vi "IRread.vi"(2 "error in (no error)":errorcluster, 3 "AI Ref In":T2) -> (0 "error out":errorcluster, 1 "紅外線數值":T1)   [LabVIEW 2019]
uses:
  <vilib>/myRIO/Instrument Drivers/Onboard IO/AI/typedefs/AI Reference.ctl
  <vilib>/myRIO/Common/Instrument Driver Framework/Utilities/typedefs/myRIO Generic Hardware Reference.ctl
  <vilib>/myRIO/Common/Instrument Driver Framework/Utilities/typedefs/Hardware Version Enum.ctl
  <vilib>/myRIO/Common/Instrument Driver Framework/Utilities/typedefs/myRIO v1.0 Reference.ctl
  <vilib>/myRIO/Common/Instrument Driver Framework/Utilities/typedefs/Generic FPGA Reference.ctl
  <vilib>/myRIO/Common/Instrument Driver Framework/myRIO v1.0/AI/typedefs/AI Channels List.ctl
  <vilib>/myRIO/Common/Instrument Driver Framework/myRIO v1.0/AI/typedefs/AI Channels Enum.ctl
  <vilib>/myRIO/Common/Instrument Driver Framework/Utilities/typedefs/Analog Scaling Constants List.ctl
  <vilib>/myRIO/Common/Instrument Driver Framework/Utilities/typedefs/Analog Scaling Constants.ctl
  <vilib>/Utility/error.llb/Error Cluster From Error Code.vi
  <vilib>/myRIO/Common/Instrument Driver Framework/myRIO v1.0/AI/vis/myRIO v1.0 Read AI.vi
  <vilib>/myRIO/Instrument Drivers/Onboard IO/AI/AI.lvlib
  <vilib>/ptbypt/NI_PtbyPt.lvlib
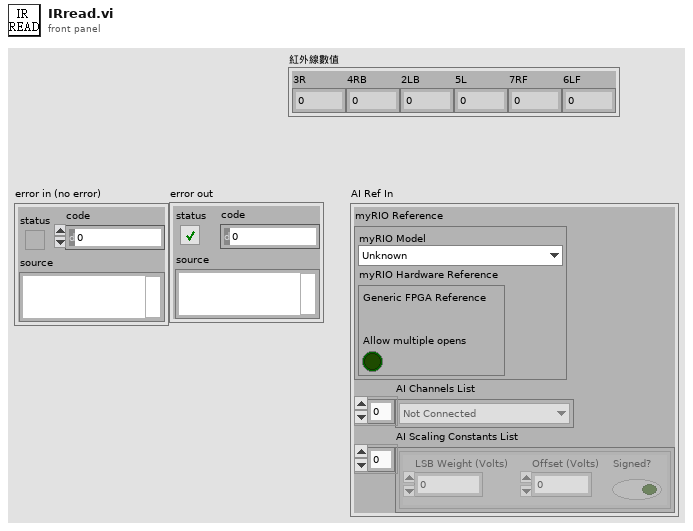
[diagram p1: front panel]
types:
  T1 = cluster{"7RF":dbl, "3R":dbl, "4RB":dbl, "5L":dbl, "6LF":dbl, "2LB":dbl}
  T2 = typedef "AI.lvlib/AI Reference.ctl" = cluster{"myRIO Reference":T3, "AI Channels List":T7, "AI Scaling Constants List":T9}
  T3 = typedef "myRIO Generic Hardware Reference.ctl" = cluster{"myRIO Model":T4, "myRIO Hardware Reference":T5}
  T4 = typedef "Hardware Version Enum.ctl" = enum16{"Unknown", "myRIO-1900", "myRIO-1950", "roboRIO", "NI ELVIS RIO CM", "ELVIS III"}
  T5 = typedef "myRIO v1.0 Reference.ctl" = cluster{"Generic FPGA Reference":T6, "Allow multiple opens":bool}
  T6 = typedef "Generic FPGA Reference.ctl" = refnum<k20>
  T7 = typedef "AI Channels List.ctl" = T8[]
  T8 = typedef "AI Channels Enum.ctl" = enum16{"Not Connected", "AudioIn/Left", "AudioIn/Right", "C/AI0", "C/AI1", "A/AI0", "A/AI1", "A/AI2", "A/AI3", "A/AI4", "A/AI5", "A/AI6", "A/AI7", "B/AI0", "B/AI1", "B/AI2", "B/AI3", "B/AI4", "B/AI5", "B/AI6", "B/AI7", "AI/AI0", "AI/AI1", "AI/AI2", "AI/AI3", "A/AI0 (DIFF)", "A/AI1 (DIFF)", "A/AI2 (DIFF)", "A/AI3 (DIFF)", "B/AI0 (DIFF)", "B/AI1 (DIFF)", "B/AI2 (DIFF)", "B/AI3 (DIFF)"}
  T9 = typedef "Analog Scaling Constants List.ctl" = T10[]
  T10 = typedef "Analog Scaling Constants.ctl" = cluster{"LSB Weight (Volts)":dbl, "Offset (Volts)":dbl, "Signed?":bool}
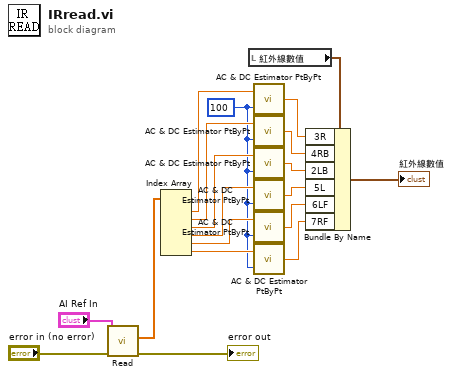
[diagram p0: block diagram]
diagram:
  w1 = 100 ("sample length")
  n1 = call <vilib>:"Read.vi"("error in (no error)"="error in (no error)", "AI Ref In"="AI Ref In") -> ("error out"=→"error out":errorcluster, "Values"=w18:dbl[])  [unwired: 7 in, 1 out]
  n2 = Index Array(array=w18) -> (element #1=w13:dbl, element #2=w12:dbl, element #3=w11:dbl, element #4=w10:dbl, element #5=w9:dbl, element #6=w8:dbl)  [unwired: 6 in]
  n3 = local read "紅外線數值"() -> (w14:T1)
  n4 = call <vilib>:"AC & DC Estimator PtByPt.vi"("signal"=w13, "sample length"=w1) -> ("DC estimate (V)"=w7:dbl)  [unwired: 1 in, 2 out]
  n5 = call <vilib>:"AC & DC Estimator PtByPt.vi"("signal"=w12, "sample length"=w1) -> ("DC estimate (V)"=w6:dbl)  [unwired: 1 in, 2 out]
  n6 = call <vilib>:"AC & DC Estimator PtByPt.vi"("signal"=w11, "sample length"=w1) -> ("DC estimate (V)"=w5:dbl)  [unwired: 1 in, 2 out]
  n7 = call <vilib>:"AC & DC Estimator PtByPt.vi"("signal"=w10, "sample length"=w1) -> ("DC estimate (V)"=w4:dbl)  [unwired: 1 in, 2 out]
  n8 = call <vilib>:"AC & DC Estimator PtByPt.vi"("signal"=w9, "sample length"=w1) -> ("DC estimate (V)"=w3:dbl)  [unwired: 1 in, 2 out]
  n9 = call <vilib>:"AC & DC Estimator PtByPt.vi"("signal"=w8, "sample length"=w1) -> ("DC estimate (V)"=w2:dbl)  [unwired: 1 in, 2 out]
  n10 = Bundle By Name(cluster=w14, "3R"=w7, "4RB"=w6, "2LB"=w5, "5L"=w4, "6LF"=w3, "7RF"=w2) -> (→"紅外線數值":T1)
